vi "Close.vi"(8 "error in (no error)":errorcluster, 11 "ToastSource in":refnum<class "ToastSource.lvclass">) -> (0 "error out":errorcluster)   [LabVIEW 2026, in "ToastNotification.lvlib" / "ToastSource.lvclass"]
doc: "Dynamic cleanup operation for a caller-owned ToastSource. The base method owns no resource and performs no action, with or without incoming error; it propagates the error. Concrete implementations must attempt cleanup even on incoming error and preserve the primary error. No source output is returned. ToastService.Close does not close this source."
uses:
  ToastSource.lvclass
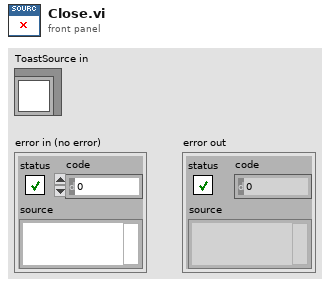
[diagram p1: front panel]
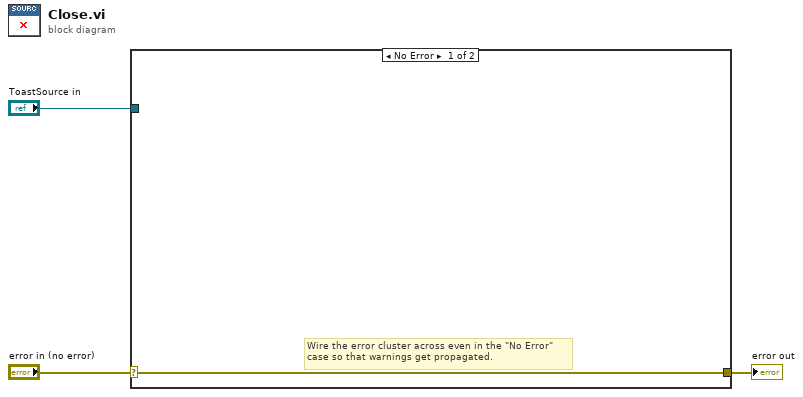
[diagram p0: block diagram]
diagram:
  n1 = case shown="No Error" "error in (no error)" {
    selector: "error in (no error)" -> [w4 w5]
    tunnel: [w4 w5] -> w2
    tunnel: "ToastSource in" -> [_ _]
    frame No Error {
      # "Wire the error cluster across even in the \"No Error\"\ncase so that warnings get propagated."
    }
    frame Error {
    }
  }
  "error out" <- w2
